vi "Short and Filter Table.vi"(5 "Sort By Ref":refnum<vi>, 6 "Headers":string[](array[string]), 7 "Filter String Ref":refnum<vi>, 8 "error in":errorcluster, 10 "Table Ref":refnum<vi>, 11 "Table Data":string[][](array[string])) -> (0 "error out":errorcluster, 3 "Sorted Table Data out":string[][](array[string]))   [LabVIEW 2025, in "Automotive Ethernet Bus Monitor UI.lvlib"]
doc: "Short and Filter the data based on the Short By and Filter Inputs, when this functionality is not paused."
uses:
  Automotive Ethernet Bus Monitor UI.lvlib
  Table_Filtering/Table_Filtering.lvlib
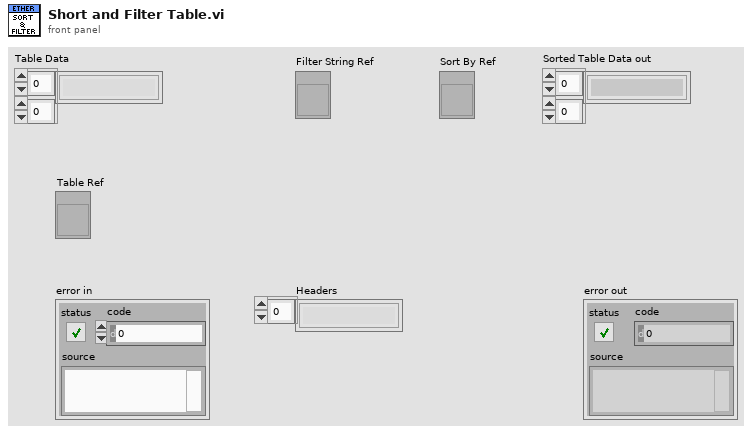
[diagram p1: front panel]
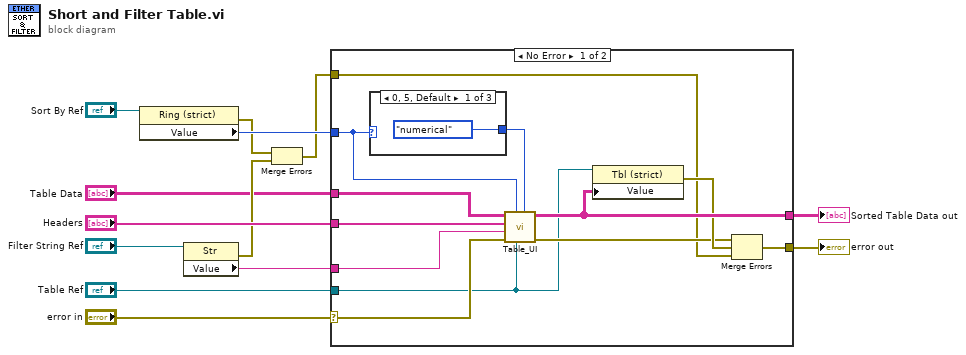
[diagram p0: block diagram]
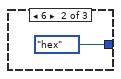
[diagram p2: hidden frame]
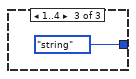
[diagram p3: hidden frame]
diagram:
  n1 = property class="Ring (strict)"(reference="Sort By Ref") -> (error out=w5:errorcluster, "Value"=w6:u16)  [unwired: 1 in, 1 out]
  n2 = property class="Str"(reference="Filter String Ref") -> (error out=w2:errorcluster, "Value"=w7:string)  [unwired: 1 in, 1 out]
  n3 = Merge Errors(w5, w2) -> (w3:errorcluster)
  n4 = case shown="No Error" "error in" {
    selector: "error in" -> [w24 w30]
    tunnel: w6 -> [w25 _]
    tunnel: w7 -> [w22 _]
    tunnel: "Headers" -> [w21 _]
    tunnel: [w20 w30] -> w4
    tunnel: "Table Ref" -> [w15 _]
    tunnel: [w23 w29] -> w10
    tunnel: w3 -> [w16 _]
    tunnel: "Table Data" -> [w14 w29]
    frame No Error {
      n5 = case shown="0, 5, Default" w25 {
        tunnel: [enum16{"numerical", "hex", "string"}."numerical" ("Sort Type") enum16{"numerical", "hex", "string"}."hex" ("Sort Type") enum16{"numerical", "hex", "string"}."string" ("Sort Type")] -> w19
        frame 0, 5, Default {
        }
        frame 6 {
        }
        frame 1..4 {
        }
      }
      n6 = call "Table_UI.vi"("Sort Type"=w19, "Table Control"=w15, "Sort by"=w25, "error in"=w24, "Filter String"=w22, "Headers"=w21, "Unsorted Data"=w14) -> ("Error Out"=w17:errorcluster, "Table Control"=w23:string[][])  [unwired: 3 in]
      n7 = property class="Tbl (strict)"(reference=w15, "Value"=w23) -> (error out=w18:errorcluster)  [unwired: 1 in, 1 out]
      n8 = Merge Errors(w17, w18, w16) -> (w20:errorcluster)
    }
    frame Error {
    }
  }
  "error out" <- w4
  "Sorted Table Data out" <- w10
